vi "FPGA Main.vi"() -> ()   [LabVIEW 2021]
uses:
  <vilib>/rvi/Emulation/niFpgaGetClockAttributes.vi
  <vilib>/rvi/Emulation/niFpgaSctlEmulationGetInTimedLoop.vi
  <vilib>/rvi/Emulation/niFpgaEmulationReportErrorSimple.vi
  <vilib>/rvi/eio/common/nirviEmuTemplateMethod_errors.vi
  <vilib>/rvi/Emulation/niFpgaCriticalErrorInLSC.vi
  <vilib>/eio/EIONode/EIONode.xnode
panel:
  out "Mod2/CJC":fxp<+/-,24,-2>
  out "Mod2/TC3":fxp<+/-,24,-2>
  out "Mod2/TC2":fxp<+/-,24,-2>
  out "Mod2/TC1":fxp<+/-,24,-2>
  out "Mod2/TC0":fxp<+/-,24,-2>
  in  "Mod1/DIO3":bool
  out "Mod1/DIO2":bool
  out "Mod1/DIO1":bool
  out "Mod1/DIO0":bool
  out "Mod1/AI7":fxp<+,18,3>
  out "Mod1/AI6":fxp<+,18,3>
  out "Mod1/AI5":fxp<+,18,3>
  out "Mod1/AI4":fxp<+,18,3>
  out "Mod1/AI3":fxp<+,18,3>
  out "Mod1/AI2":fxp<+,18,3>
  out "Mod1/AI1":fxp<+,18,3>
  out "Mod1/AI0":fxp<+,18,3>
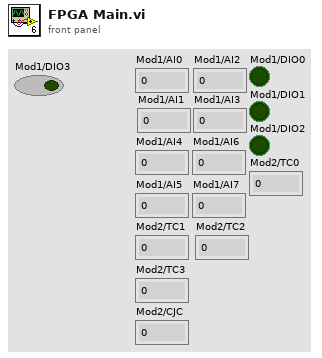
[diagram p1: front panel]
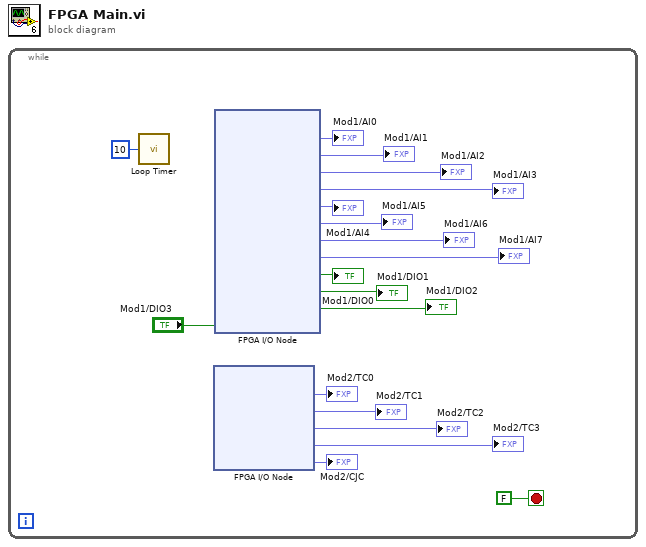
[diagram p0: block diagram]
diagram:
  n1 = while {
    stop <- FALSE stop-if-true
    n2 = call "Loop Timer"("Count(mSec)"=u32 10) -> ()  [unwired: 1 out]
    n3 = xnode "FPGA I/O Node"() -> ("Mod2/TC0"=→"Mod2/TC0":fxp<+/-,24,-2>, "Mod2/TC1"=→"Mod2/TC1":fxp<+/-,24,-2>, "Mod2/TC2"=→"Mod2/TC2":fxp<+/-,24,-2>, "Mod2/TC3"=→"Mod2/TC3":fxp<+/-,24,-2>, "Mod2/CJC"=→"Mod2/CJC":fxp<+/-,24,-2>)  [unwired: 5 in, 5 out]
    n4 = xnode "FPGA I/O Node"("Mod1/DIO3"="Mod1/DIO3") -> ("Mod1/AI0"=→"Mod1/AI0":fxp<+,18,3>, "Mod1/AI1"=→"Mod1/AI1":fxp<+,18,3>, "Mod1/AI2"=→"Mod1/AI2":fxp<+,18,3>, "Mod1/AI3"=→"Mod1/AI3":fxp<+,18,3>, "Mod1/AI4"=→"Mod1/AI4":fxp<+,18,3>, "Mod1/AI5"=→"Mod1/AI5":fxp<+,18,3>, "Mod1/AI6"=→"Mod1/AI6":fxp<+,18,3>, "Mod1/AI7"=→"Mod1/AI7":fxp<+,18,3>, "Mod1/DIO0"=→"Mod1/DIO0":bool, "Mod1/DIO1"=→"Mod1/DIO1":bool, "Mod1/DIO2"=→"Mod1/DIO2":bool)  [unwired: 12 in, 12 out]
  }
